vi "Retrieve_latest_PAQ_data.vi"(8 "error in (no error)":errorcluster, 10 "FetchLatestDefinition":T2, 11 "DBAL-BIN in":refnum<class "DBAL-BIN.lvclass">) -> (0 "error out":errorcluster, 2 "BinHistData":T1, 3 "DBAL-BIN out":refnum<class "DBAL-BIN.lvclass">)   [LabVIEW 2020, in "Sgraph_lib_V1.lvlib" / "DBAL-BIN.lvclass"]
uses:
  DBAL-BIN.lvclass
  controls/DBAL_FetchLatestFrom.ctl
  controls/BIN/BINdata.ctl
  DBAL-BIN.lvclass/DBAL-BIN.ctl
  DBAL.lvclass
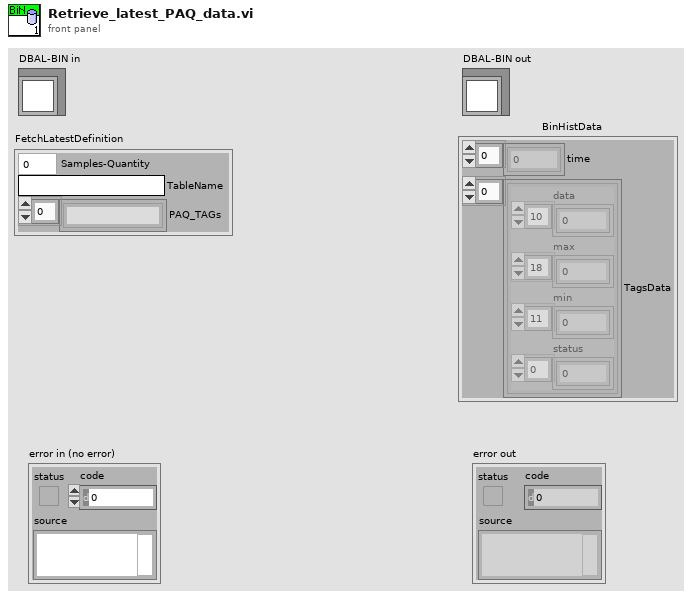
[diagram p1: front panel]
types:
  T1 = typedef "Sgraph_lib_V1.lvlib/DBAL-BIN.lvclass/BINdata.ctl" = cluster{"time":dbl[], "TagsData":cluster{"data":dbl[], "max":dbl[], "min":dbl[], "status":u32[]}[]}
  T2 = typedef "Sgraph_lib_V1.lvlib/DBAL.lvclass/DBAL_FetchLatestFrom.ctl" = cluster{"Samples-Quantity":i32, "TableName":string, "PAQ_TAGs":string[]}
  T3 = typedef "Sgraph_lib_V1.lvlib/DBAL-BIN.lvclass/BinFolderPace.ctl" = enum16{"PerDay", "PerWeek", "PerYear"}
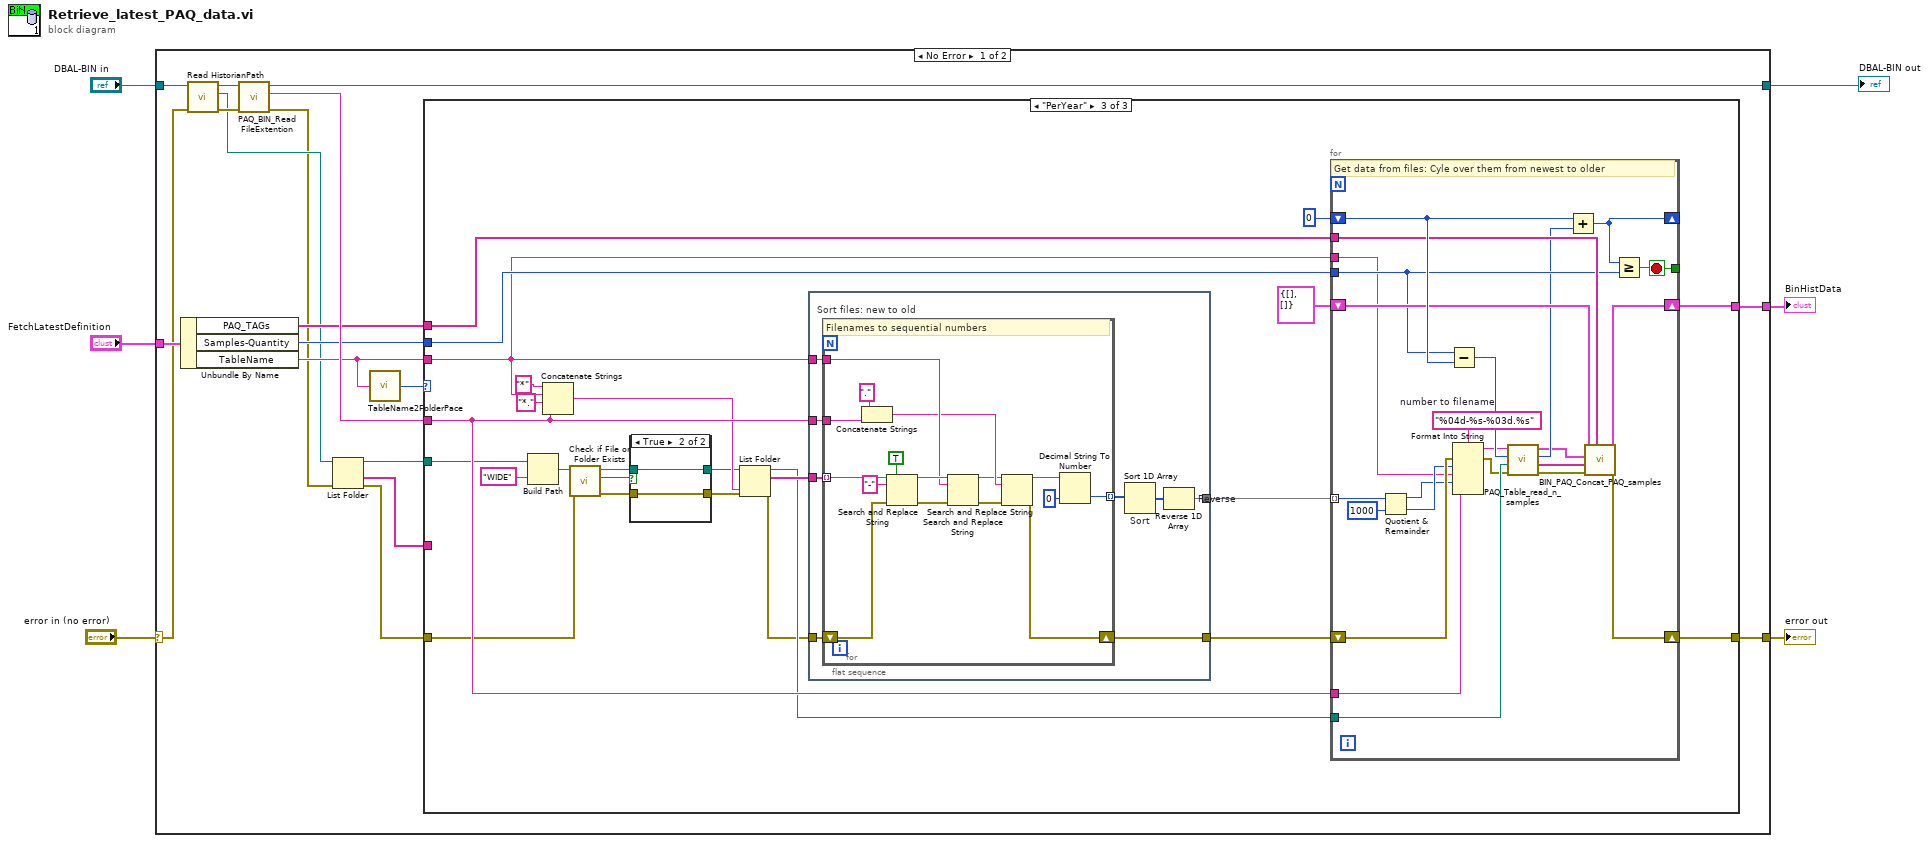
[diagram p0: block diagram]
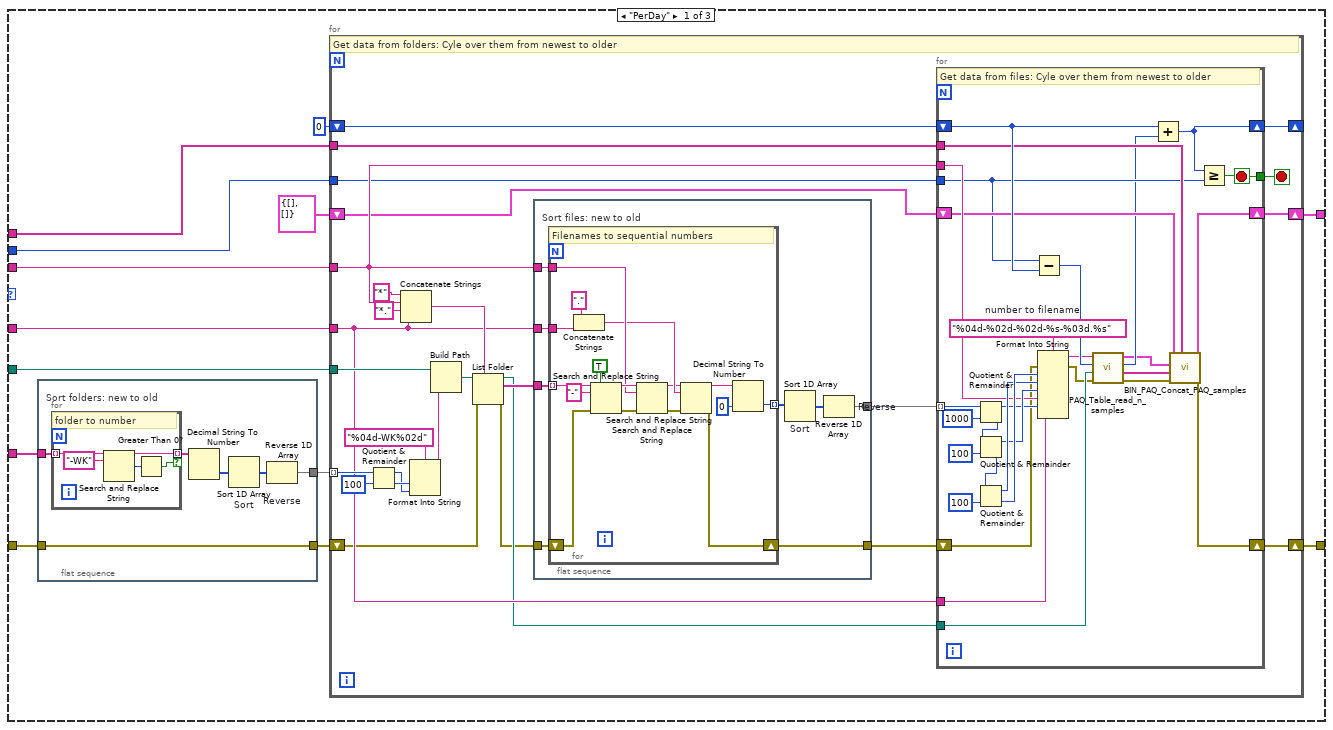
[diagram p2: hidden frame]
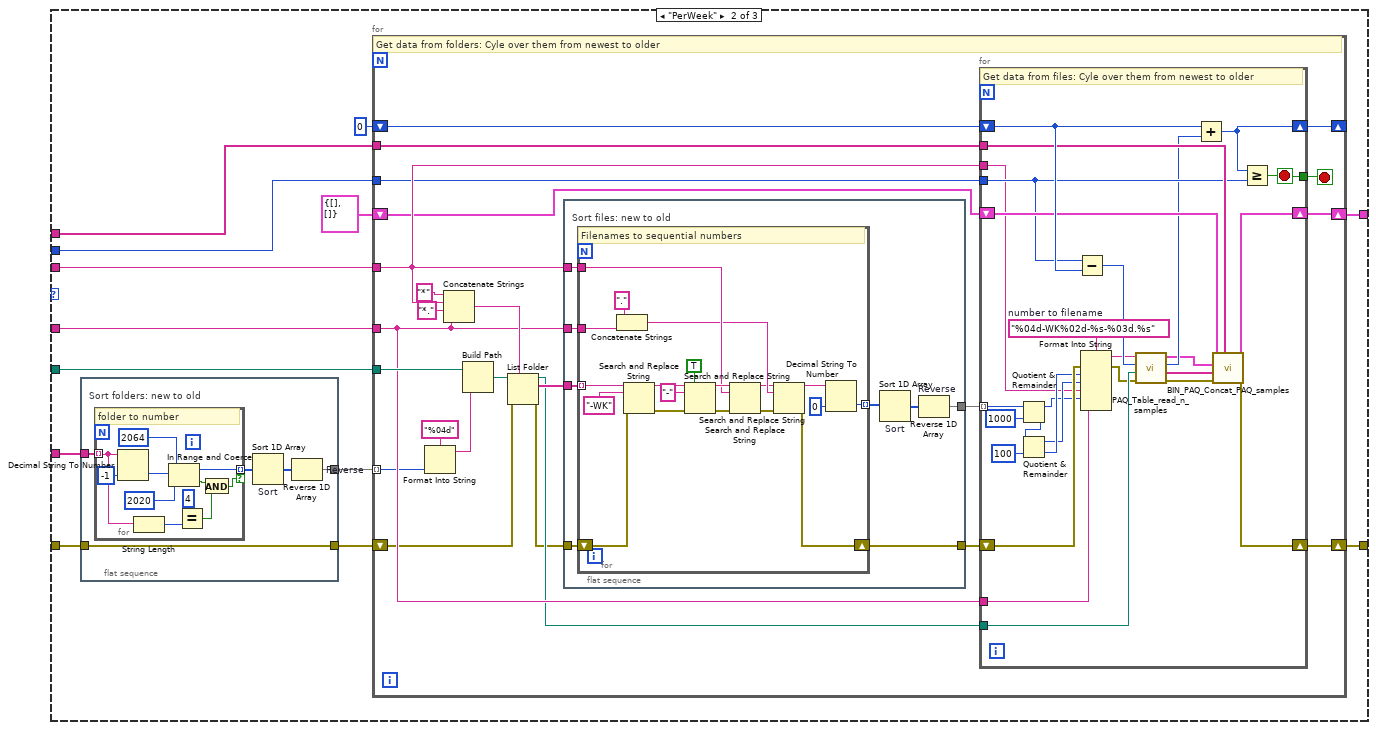
[diagram p3: hidden frame]
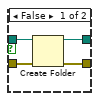
[diagram p4: hidden frame]
diagram:
  n1 = case shown="No Error" "error in (no error)" {
    selector: "error in (no error)" -> [w19 w316]
    tunnel: [w23 w316] -> w5
    tunnel: "DBAL-BIN in" -> [w20 w317]
    tunnel: [w16 w317] -> w3
    tunnel: "FetchLatestDefinition" -> [w24 _]
    tunnel: [w14 _] -> w1
    frame No Error {
      n2 = Unbundle By Name(w24) -> ("PAQ_TAGs"=w15:string[], "Samples-Quantity"=w17:i32, "TableName"=w13:string)
      n3 = call "Read HistorianPath.vi"("error in (no error)"=w19, "DBAL-BIN in"=w20) -> ("error out"=w18:errorcluster, "HistorianPath"=w11:path, "DBAL-BIN out"=w21:refnum<class "DBAL-BIN.lvclass">)  [unwired: 7 in]
      n4 = call "PAQ_BIN_Read FileExtention.vi"("error in (no error)"=w18, "DBAL-BIN in"=w21) -> ("error out"=w10:errorcluster, "FileExtention"=w22:string, "DBAL-BIN out"=w16:refnum<class "DBAL-BIN.lvclass">)  [unwired: 7 in]
      n5 = List Folder(path=w11, error in=w10) -> (path out=w7:path, folder names=w9:string[], error out=w8:errorcluster)  [unwired: 2 in, 1 out]
      n6 = call "TableName2FolderPace.vi"("TableName"=w13) -> ("FolderPace"=w12:T3)  [unwired: 6 in]
      n7 = case shown="\"PerYear\"" w12 {
        tunnel: [w37 w142 w261] -> w23
        tunnel: w22 -> [w36 w141 w260]
        tunnel: w17 -> [w35 w140 w259]
        tunnel: w15 -> [w33 w138 w258]
        tunnel: [w31 w136 w256] -> w14
        tunnel: w13 -> [w30 w135 w255]
        tunnel: w9 -> [w29 w134 _]
        tunnel: w8 -> [w27 w132 w237]
        tunnel: w7 -> [w26 w131 w254]
        frame "PerDay" {
          n8 = flat-sequence {
            tunnel: w29 -> [w43]
            tunnel: [w38] -> w25
            tunnel: w27 -> [w40]
            tunnel: [w40] -> w28
            frame #0 {
              # "Sort folders: new to old"
              n9 = for {
                tunnel: w43 -> [w48] mode=indexing
                tunnel: [w46] -> w42 mode=indexing if=w44
                # "folder to number"
                n10 = Search and Replace String(input string=w48, search string="-WK") -> (result string=w46:string, number of replacements=w45:i32)  [unwired: 6 in, 2 out]
                n11 = Greater Than 0?(x=w45) -> (x > 0?=w44:bool)
              }
              n12 = Decimal String To Number ("to num")(string=w42) -> (number=w41:i32[])  [unwired: 2 in, 1 out]
              n13 = Sort 1D Array "Sort"(array=w41) -> (sorted array=w39:i32[])
              n14 = Reverse 1D Array "Reverse"(array=w39) -> (reversed array=w38:i32[])
            }
          }
          n15 = for {
            shift-right: [w59] -> w37
            shift-left: w28 -> [w50]
            tunnel: w25 -> [w75] mode=indexing
            tunnel: w36 -> [w62]
            tunnel: w26 -> [w70]
            tunnel: w30 -> [w63]
            tunnel: w35 -> [w58]
            shift-right: [w56] -> _
            shift-left: 0 ("Fetched samples") -> [w57]
            tunnel: w33 -> [w55]
            shift-right: [w54] -> w31
            shift-left: T1 {"time"=[], "TagsData"=[]} ("BinHistData") -> [w53]
            stop <- w52 stop-if-true
            # "Get data from folders: Cyle over them from newest to older"
            n16 = Quotient & Remainder(x=w75, y=100) -> (x-y*floor(x/y)=w71:i32, floor(x/y)=w72:i32)
            n17 = Concatenate Strings("*", w63, "*.", w62) -> (w66:string)
            n18 = Format Into String(format string="%04d-WK%02d", w72, w71) -> (resulting string=w51:string)  [unwired: 2 in, 1 out]
            n19 = Build Path(base path=w70, name or relative path=w51) -> (appended path=w69:path)
            n20 = List Folder(path=w69, pattern=w66, error in=w50) -> (path out=w61:path, filenames=w64:string[], error out=w49:errorcluster)  [unwired: 1 in, 1 out]
            n21 = flat-sequence {
              tunnel: w64 -> [w113]
              tunnel: w63 -> [w112]
              tunnel: w62 -> [w111]
              tunnel: [w108] -> w65
              tunnel: w49 -> [w107]
              tunnel: [w106] -> w60
              frame #0 {
                # "Sort files: new to old"
                n22 = for {
                  tunnel: w113 -> [w118] mode=indexing
                  tunnel: w112 -> [w126]
                  tunnel: w111 -> [w125]
                  tunnel: [w120] -> w109 mode=indexing
                  shift-right: [w114] -> w106
                  shift-left: w107 -> [w117]
                  # "Filenames to sequential numbers"
                  n23 = Concatenate Strings("." ("string"), w125) -> (w124:string)
                  n24 = Search and Replace String(replace all?=TRUE ("replace all? (F)"), input string=w118, search string="-", error in=w117) -> (result string=w127:string, error out=w116:errorcluster)  [unwired: 4 in, 2 out]
                  n25 = Search and Replace String(input string=w127, search string=w126, error in=w116) -> (result string=w123:string, error out=w115:errorcluster)  [unwired: 5 in, 2 out]
                  n26 = Search and Replace String(input string=w123, search string=w124, error in=w115) -> (result string=w121:string, error out=w114:errorcluster)  [unwired: 5 in, 2 out]
                  n27 = Decimal String To Number(string=w121, default (0L)=u64 0 ("default (0 I32)")) -> (number=w120:u64)  [unwired: 1 in, 1 out]
                }
                n28 = Sort 1D Array "Sort"(array=w109) -> (sorted array=w110:u64[])
                n29 = Reverse 1D Array "Reverse"(array=w110) -> (reversed array=w108:u64[])
              }
            }
            n30 = for {
              tunnel: w65 -> [w104] mode=indexing
              tunnel: w63 -> [w95]
              tunnel: w62 -> [w93]
              tunnel: w61 -> [w91]
              shift-right: [w84] -> w59
              shift-left: w60 -> [w92]
              tunnel: w58 -> [w81]
              shift-right: [w77] -> w56
              shift-left: w57 -> [w88]
              tunnel: w55 -> [w82]
              shift-right: [w86] -> w54
              shift-left: w53 -> [w87]
              tunnel: [w80] -> w52
              stop <- w80 stop-if-true
              w99 = "%04d-%02d-%02d-%s-%03d.%s"  # number to filename
              # "Get data from files: Cyle over them from newest to older"
              n31 = Quotient & Remainder(x=w104, y=u64 1000) -> (x-y*floor(x/y)=w94:u64, floor(x/y)=w102:u64)
              n32 = Quotient & Remainder(x=w102, y=u64 100) -> (x-y*floor(x/y)=w96:u64, floor(x/y)=w100:u64)
              n33 = Quotient & Remainder(x=w100, y=u64 100) -> (x-y*floor(x/y)=w97:u64, floor(x/y)=w98:u64)
              n34 = Subtract(x=w81, y=w88) -> (x-y=w89:i32)
              n35 = Format Into String(format string=w99, error in=w92, w98, w97, w96, w95, w94, w93) -> (resulting string=w76:string, error out=w90:errorcluster)  [unwired: 1 in]
              n36 = call "PAQ_Table_read_n_samples.vi"("error in (no error)"=w90, "Sub Path"=w91, "Required samples"=w89, "Table Filename"=w76) -> ("error out"=w85:errorcluster, "TAGs"=w83:string[], "Fetched samples"=w79:i32, "value"=w78:T1)  [unwired: 4 in]
              n37 = Add(x=w88, y=w79) -> (x+y=w77:i32)
              n38 = call "BIN_PAQ_Concat_PAQ_samples.vi"("Memory TAGs"=w82, "error in (no error)"=w85, "Added samples TAGs"=w83, "PAQ Samples to ADD"=w78, "PAQ Samples IN"=w87) -> ("error out"=w84:errorcluster, "PAQ Samples OUT"=w86:T1)  [unwired: 5 in]
              n39 = Greater Or Equal?(x=w77, y=w81) -> (x >= y?=w80:bool)
            }
          }
        }
        frame "PerWeek" {
          n40 = flat-sequence {
            tunnel: w134 -> [w147]
            tunnel: [w144] -> w130
            tunnel: w132 -> [w146]
            tunnel: [w146] -> w133
            frame #0 {
              # "Sort folders: new to old"
              n41 = for {
                tunnel: w147 -> [w153] mode=indexing
                tunnel: [w154] -> w143 mode=indexing if=w148
                # "folder to number"
                n42 = Decimal String To Number ("to num")(string=w153, default (0L)=-1 ("default (0 I32)")) -> (number=w157:i32)  [unwired: 1 in, 1 out]
                n43 = String Length(string=w153) -> (length=w152:i32)
                n44 = In Range and Coerce(upper limit=2064 ("lower limit"), x=w157, lower limit=2020) -> (coerced(x)=w154:i32, In Range?=w150:bool)
                n45 = Equal?(x=4, y=w152) -> (x = y?=w149:bool)
                n46 = And(x=w150, y=w149) -> (x .and. y?=w148:bool)
              }
              n47 = Sort 1D Array "Sort"(array=w143) -> (sorted array=w145:i32[])
              n48 = Reverse 1D Array "Reverse"(array=w145) -> (reversed array=w144:i32[])
            }
          }
          n49 = for {
            shift-right: [w170] -> w142
            shift-left: w133 -> [w160]
            tunnel: w130 -> [w161] mode=indexing
            tunnel: w141 -> [w173]
            tunnel: w131 -> [w181]
            tunnel: w135 -> [w174]
            tunnel: w140 -> [w169]
            shift-right: [w167] -> _
            shift-left: 0 ("Fetched samples") -> [w168]
            tunnel: w138 -> [w166]
            shift-right: [w165] -> w136
            shift-left: T1 {"time"=[], "TagsData"=[]} ("BinHistData") -> [w164]
            stop <- w163 stop-if-true
            # "Get data from folders: Cyle over them from newest to older"
            n50 = Format Into String(format string="%04d", w161) -> (resulting string=w162:string)  [unwired: 2 in, 1 out]
            n51 = Concatenate Strings("*", w174, "*.", w173) -> (w177:string)
            n52 = Build Path(base path=w181, name or relative path=w162) -> (appended path=w180:path)
            n53 = List Folder(path=w180, pattern=w177, error in=w160) -> (path out=w172:path, filenames=w175:string[], error out=w159:errorcluster)  [unwired: 1 in, 1 out]
            n54 = flat-sequence {
              tunnel: w175 -> [w217]
              tunnel: w174 -> [w216]
              tunnel: w173 -> [w215]
              tunnel: [w212] -> w176
              tunnel: w159 -> [w211]
              tunnel: [w210] -> w171
              frame #0 {
                # "Sort files: new to old"
                n55 = for {
                  tunnel: w217 -> [w226] mode=indexing
                  tunnel: w216 -> [w234]
                  tunnel: w215 -> [w233]
                  tunnel: [w228] -> w213 mode=indexing
                  shift-right: [w218] -> w210
                  shift-left: w211 -> [w222]
                  # "Filenames to sequential numbers"
                  n56 = Concatenate Strings("." ("string"), w233) -> (w232:string)
                  n57 = Search and Replace String(input string=w226, search string="-WK", error in=w222) -> (result string=w224:string, error out=w221:errorcluster)  [unwired: 5 in, 2 out]
                  n58 = Search and Replace String(replace all?=TRUE ("replace all? (F)"), input string=w224, search string="-", error in=w221) -> (result string=w235:string, error out=w220:errorcluster)  [unwired: 4 in, 2 out]
                  n59 = Search and Replace String(input string=w235, search string=w234, error in=w220) -> (result string=w231:string, error out=w219:errorcluster)  [unwired: 5 in, 2 out]
                  n60 = Search and Replace String(input string=w231, search string=w232, error in=w219) -> (result string=w229:string, error out=w218:errorcluster)  [unwired: 5 in, 2 out]
                  n61 = Decimal String To Number(string=w229, default (0L)=u64 0 ("default (0 I32)")) -> (number=w228:u64)  [unwired: 1 in, 1 out]
                }
                n62 = Sort 1D Array "Sort"(array=w213) -> (sorted array=w214:u64[])
                n63 = Reverse 1D Array "Reverse"(array=w214) -> (reversed array=w212:u64[])
              }
            }
            n64 = for {
              tunnel: w176 -> [w208] mode=indexing
              tunnel: w174 -> [w186]
              tunnel: w173 -> [w184]
              tunnel: w172 -> [w203]
              shift-right: [w196] -> w170
              shift-left: w171 -> [w204]
              tunnel: w169 -> [w193]
              shift-right: [w189] -> w167
              shift-left: w168 -> [w200]
              tunnel: w166 -> [w194]
              shift-right: [w198] -> w165
              shift-left: w164 -> [w199]
              tunnel: [w192] -> w163
              stop <- w192 stop-if-true
              w205 = "%04d-WK%02d-%s-%03d.%s"  # number to filename
              # "Get data from files: Cyle over them from newest to older"
              n65 = Quotient & Remainder(x=w208, y=u64 1000) -> (x-y*floor(x/y)=w185:u64, floor(x/y)=w206:u64)
              n66 = Quotient & Remainder(x=w206, y=u64 100) -> (x-y*floor(x/y)=w187:u64, floor(x/y)=w188:u64)
              n67 = Subtract(x=w193, y=w200) -> (x-y=w201:i32)
              n68 = Format Into String(format string=w205, error in=w204, w188, w187, w186, w185, w184) -> (resulting string=w183:string, error out=w202:errorcluster)  [unwired: 1 in]
              n69 = call "PAQ_Table_read_n_samples.vi"("error in (no error)"=w202, "Sub Path"=w203, "Required samples"=w201, "Table Filename"=w183) -> ("error out"=w197:errorcluster, "TAGs"=w195:string[], "Fetched samples"=w191:i32, "value"=w190:T1)  [unwired: 4 in]
              n70 = Add(x=w200, y=w191) -> (x+y=w189:i32)
              n71 = call "BIN_PAQ_Concat_PAQ_samples.vi"("Memory TAGs"=w194, "error in (no error)"=w197, "Added samples TAGs"=w195, "PAQ Samples to ADD"=w190, "PAQ Samples IN"=w199) -> ("error out"=w196:errorcluster, "PAQ Samples OUT"=w198:T1)  [unwired: 5 in]
              n72 = Greater Or Equal?(x=w189, y=w193) -> (x >= y?=w192:bool)
            }
          }
        }
        frame "PerYear" {
          n73 = Build Path(base path=w254, name or relative path="WIDE" ("format string")) -> (appended path=w243:path)
          n74 = Concatenate Strings("*", w255, "*.", w260) -> (w251:string)
          n75 = call <vilib>:"Check if File or Folder Exists.vi"("error in (no error)"=w237, "path"=w243) -> ("error out"=w239:errorcluster, "file or folder exists?"=w242:bool, "dup path"=w241:path)  [unwired: 7 in]
          n76 = case shown="True" w242 {
            tunnel: w241 -> [w265 w267]
            tunnel: [w262 w267] -> w240
            tunnel: w239 -> [w264 w266]
            tunnel: [w263 w266] -> w238
            frame False {
              n77 = Create Folder(path (use dialog)=w265, error in=w264) -> (created path=w262:path, error out=w263:errorcluster)  [unwired: 1 in, 1 out]
            }
            frame True {
            }
          }
          n78 = List Folder(path=w240, pattern=w251, error in=w238) -> (path out=w248:path, filenames=w249:string[], error out=w244:errorcluster)  [unwired: 1 in, 1 out]
          n79 = flat-sequence {
            tunnel: w249 -> [w299]
            tunnel: w255 -> [w298]
            tunnel: w260 -> [w297]
            tunnel: [w294] -> w250
            tunnel: w244 -> [w293]
            tunnel: [w292] -> w247
            frame #0 {
              # "Sort files: new to old"
              n80 = for {
                tunnel: w299 -> [w300] mode=indexing
                tunnel: w298 -> [w313]
                tunnel: w297 -> [w312]
                tunnel: [w307] -> w295 mode=indexing
                shift-right: [w302] -> w292
                shift-left: w293 -> [w301]
                # "Filenames to sequential numbers"
                n81 = Concatenate Strings("." ("string"), w312) -> (w311:string)
                n82 = Search and Replace String(replace all?=TRUE ("replace all? (F)"), input string=w300, search string="-", error in=w301) -> (result string=w314:string, error out=w304:errorcluster)  [unwired: 4 in, 2 out]
                n83 = Search and Replace String(input string=w314, search string=w313, error in=w304) -> (result string=w310:string, error out=w303:errorcluster)  [unwired: 5 in, 2 out]
                n84 = Search and Replace String(input string=w310, search string=w311, error in=w303) -> (result string=w308:string, error out=w302:errorcluster)  [unwired: 5 in, 2 out]
                n85 = Decimal String To Number(string=w308, default (0L)=u64 0 ("default (0 I32)")) -> (number=w307:u64)  [unwired: 1 in, 1 out]
              }
              n86 = Sort 1D Array "Sort"(array=w295) -> (sorted array=w296:u64[])
              n87 = Reverse 1D Array "Reverse"(array=w296) -> (reversed array=w294:u64[])
            }
          }
          n88 = for {
            tunnel: w250 -> [w290] mode=indexing
            tunnel: w255 -> [w270]
            tunnel: w260 -> [w268]
            tunnel: w248 -> [w287]
            shift-right: [w280] -> w261
            shift-left: w247 -> [w288]
            tunnel: w259 -> [w277]
            shift-right: [w273] -> _
            shift-left: 0 ("Fetched samples") -> [w284]
            tunnel: w258 -> [w278]
            shift-right: [w282] -> w256
            shift-left: T1 {"time"=[], "TagsData"=[]} ("BinHistData") -> [w283]
            tunnel: [w276] -> _
            stop <- w276 stop-if-true
            w289 = "%04d-%s-%03d.%s"  # number to filename
            # "Get data from files: Cyle over them from newest to older"
            n89 = Quotient & Remainder(x=w290, y=u64 1000) -> (x-y*floor(x/y)=w269:u64, floor(x/y)=w271:u64)
            n90 = Subtract(x=w277, y=w284) -> (x-y=w285:i32)
            n91 = Format Into String(format string=w289, error in=w288, w271, w270, w269, w268) -> (resulting string=w272:string, error out=w286:errorcluster)  [unwired: 1 in]
            n92 = call "PAQ_Table_read_n_samples.vi"("error in (no error)"=w286, "Sub Path"=w287, "Required samples"=w285, "Table Filename"=w272) -> ("error out"=w281:errorcluster, "TAGs"=w279:string[], "Fetched samples"=w275:i32, "value"=w274:T1)  [unwired: 4 in]
            n93 = Add(x=w284, y=w275) -> (x+y=w273:i32)
            n94 = call "BIN_PAQ_Concat_PAQ_samples.vi"("Memory TAGs"=w278, "error in (no error)"=w281, "Added samples TAGs"=w279, "PAQ Samples to ADD"=w274, "PAQ Samples IN"=w283) -> ("error out"=w280:errorcluster, "PAQ Samples OUT"=w282:T1)  [unwired: 5 in]
            n95 = Greater Or Equal?(x=w273, y=w277) -> (x >= y?=w276:bool)
          }
        }
      }
    }
    frame Error {
    }
  }
  "error out" <- w5
  "DBAL-BIN out" <- w3
  "BinHistData" <- w1
